vi "Documentation.vi"() -> (0 "Author":string, 1 "History":string, 2 "Version":string, 3 "Description":string)   [LabVIEW 2021, in "CAN_Writer_NIXNET_Plugin.lvlib"]
uses:
  CAN_Writer_NIXNET_Plugin.lvlib
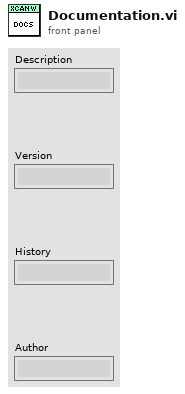
[diagram p1: front panel]
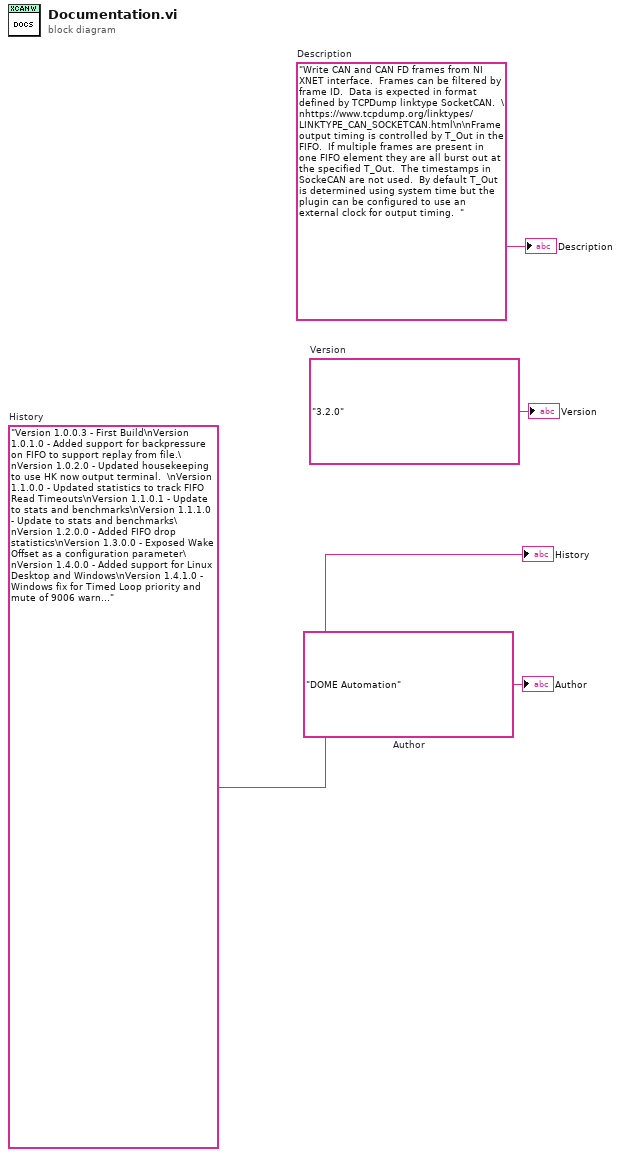
[diagram p0: block diagram]
diagram:
  w1 = "DOME Automation"  # Author
  w2 = "Version 1.0.0.3 - First Build\nVersion 1.0.1.0 - Added support for backpressure on FIFO to support replay from file.\nVersion 1.0.2.0 - Updated housekeeping to use HK now output terminal.  \nVersion 1.1.0.0 - Updated statistics to track FIFO Read Timeouts\nVersion 1.1.0.1 - Update to stats and benchmarks\nVersion 1.1.1.0 - Update to stats and benchmarks\nVersion 1.2.0.0 - Added FIFO drop statistics\nVersion 1.3.0.0 - Exposed Wake Offset as a configuration parameter\nVersion 1.4.0.0 - Added support for Linux Desktop and Windows\nVersion 1.4.1.0 - Windows fix for Timed Loop priority and mute of 9006 warning.  \nVersion 1.4.2.0 - Windows Log timestamp update to use wall clock time\nVersion 1.4.3.0 - Standard support for mute late cycle warnings on Linux and Windows.  Mute gRCP client timeout in UI.\nVersion 1.4.4.0 - Flexible tag linking support added.\nVersion 2.0.0.0 - Update to gRPC core library.\nVersion 2.0.1.0 - Support for Core UI Class update\nVersion 2.0.2.0 - Register gRPC Descriptors set as config option\nVersion 3.0.0.0 - Support for Core Class to Events\nVersion 3.0.1.0 - Include updated CIPC with bug fix for backpressure and Core update with bug fix to handle error from cleanup.\nVersion 3.0.2.0 - Incorporate core update to close plugin on disconnect of CIF manager\nVersion 3.0.4.0 - Memory optimization\nVersion 3.0.5.0 - Incorporate LV gRPC core library updates to fix memory leaks\nVersion 3.1.0.0 - Support for \"one shot\" write configuration where no ack will not fault the plugin\rVersion 3.2.0.0 - Added support for CAN Status monitoring and improved error on faults."  # History
  w3 = "3.2.0"  # Version
  w4 = "Write CAN and CAN FD frames from NI XNET interface.  Frames can be filtered by frame ID.  Data is expected in format defined by TCPDump linktype SocketCAN.  \nhttps://www.tcpdump.org/linktypes/LINKTYPE_CAN_SOCKETCAN.html\n\nFrame output timing is controlled by T_Out in the FIFO.  If multiple frames are present in one FIFO element they are all burst out at the specified T_Out.  The timestamps in SockeCAN are not used.  By default T_Out is determined using system time but the plugin can be configured to use an external clock for output timing.  "  # Description
  "Description" <- w4
  "Version" <- w3
  "History" <- w2
  "Author" <- w1
